vi "Initialize.vi"(2 "XRef":refnum<vi>) -> (1 "State Out":T1)   [LabVIEW 2012, in "Minimum Array Size.xnode"]
uses:
  Minimum Array Size.xnode
  State.ctl
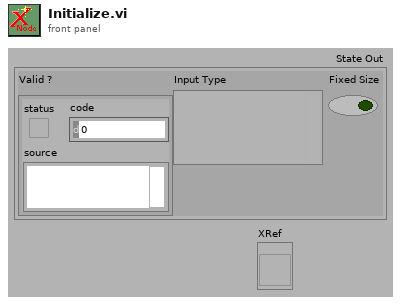
[diagram p1: front panel]
types:
  T1 = typedef "Minimum Array Size.xnode/State.ctl" = cluster{"Valid ?":errorcluster, "Input Type":variant, "Fixed Size":bool}
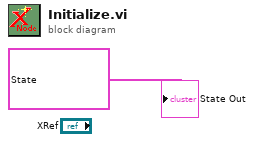
[diagram p0: block diagram]
diagram:
  "State Out" <- T1 {"Valid ?"={"status"=TRUE, "code"=-1, "source"="Initialised"}, "Input Type"=variant, "Fixed Size"=FALSE} ("State Out")
